vi "RemoteVI Start.vi"(0 "VI":refnum<vi>, 1 "whole network?":bool, 2 "token":string, 3 "view only?":bool, 5 "port":u16=8088, 7 "fps":dbl=20.0, 11 "error in":errorcluster) -> (4 "URL":string, 15 "error out":errorcluster)   [LabVIEW 2020, in "RemoteVI.lvlib"]
doc: "Shares the front panel of VI in a web browser and returns immediately. Leave VI unwired to share the CALLER (the VI one level up in the call chain, opened by name). URL is the link to open, with the share's access token: every request needs it (docs\\security.md). By default the share is reachable from this computer only (http://127.0.0.1:<port>/?t=...); whole network? TRUE listens on every interface and the URL uses this computer's IP address. token empty makes a new random token (32 hex digits from the operating system's secure random number generator); view only? TRUE ignores the browsers' input. Several shares can run in one LabVIEW application instance, each on its own port (the Server Loop is reentrant): a port that is already shared here returns error 5001 and launches nothing. Otherwise (RemoteVI Launch Share.vi) Start opens a new clone of ..\\Server\\RemoteVI Server Loop.vi (RemoteVI Open Server Loop.vi), sets its controls and runs it without waiting (RemoteVI Launch Server Loop.vi), and waits until the loop has created its TCP listener: the loop sends the listener's error cluster on the notifier RemoteVI:<port>:started, and Start returns that error (e.g. 60 when the port is in use - the loop has then already ended), or 5002 when nothing arrives within 2 s. So error out is clean only when the panel is being served. The share stops on RemoteVI Stop.vi with the same port, or by itself once VI is no longer running. RemoteVI Status.vi tells what is shared."
uses:
  RemoteVI.lvlib
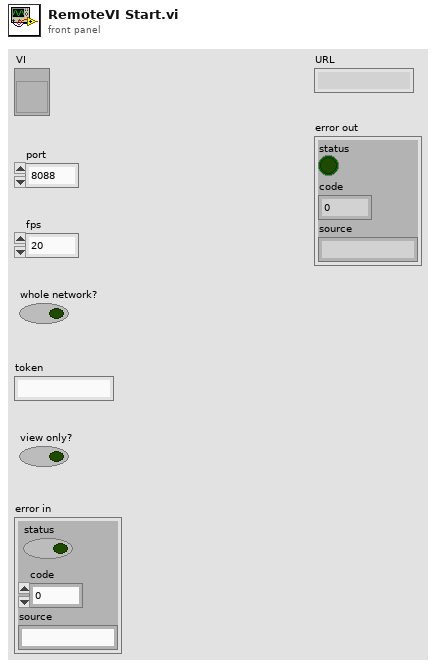
[diagram p1: front panel]
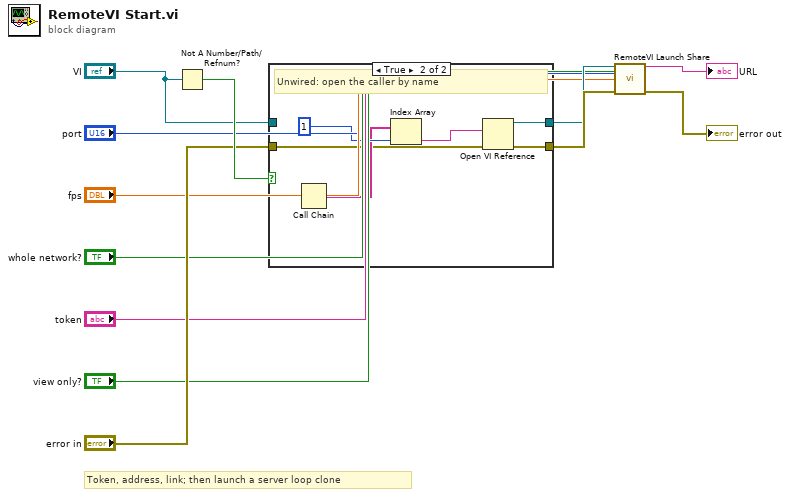
[diagram p0: block diagram]
diagram:
  # "Token, address, link; then launch a server loop clone"
  n1 = Not A Number/Path/Refnum?(number/path/refnum="VI") -> (NaN/Path/Refnum?=w8:bool)
  n2 = case shown="True" w8 {
    tunnel: "VI" -> [w13 _]
    tunnel: "error in" -> [w14 w15]
    tunnel: [w13 w19] -> w9
    tunnel: [w14 w20] -> w10
    frame False {
    }
    frame True {
      # "Unwired: open the caller by name"
      n3 = Call Chain() -> (call chain=w16:string[])
      n4 = Index Array(array=w16, index=1) -> (element=w18:string)
      n5 = Open VI Reference(vi path=w18, error in (no error)=w15) -> (vi reference=w19:refnum<vi>, error out=w20:errorcluster)  [unwired: 4 in]
    }
  }
  n6 = call "RemoteVI Launch Share.vi"("VI"=w9, "whole network?"="whole network?", "token"="token", "view only?"="view only?", "port"="port", "fps"="fps", "error in"=w10) -> ("URL"=→"URL":string, "error out"=→"error out":errorcluster)  [unwired: 7 in]
